vi "Digit to Color Converter.vi"(4 "Digit select":T1) -> (1 "Digit Color":u32(colorbox))   [LabVIEW 2018, in "Resistance Colors.lvlib"]
doc: "Converts the selected Digit Enum value into the corresponding color for the resistor band.\n\nThe VI receives the <b>Digit select</b> input and returns the corresponding resistor band color through <b>Digit Color</b>.\n\nThe color is determined by mapping the selected Enum item to the corresponding color constant."
uses:
  Resistance Colors.lvlib
  Resistor Controls/Digit--enum.ctl
  Band Colors/Band Colors.lvlib
  Resistor Controls/Resistance Controls.lvlib
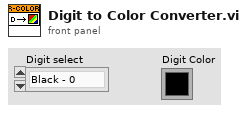
[diagram p1: front panel]
types:
  T1 = typedef "Resistance Controls.lvlib/Digit--enum.ctl" = enum16{"Black - 0", "Brown - 1", "Red - 2", "Orange - 3", "Yellow - 4", "Green - 5", "Blue - 6", "Violet - 7", "Grey - 8", "White - 9"}
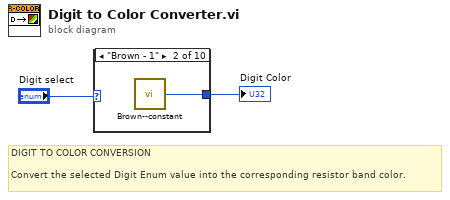
[diagram p0: block diagram]
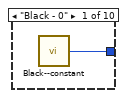
[diagram p2: hidden frame]
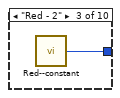
[diagram p3: hidden frame]
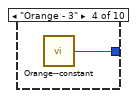
[diagram p4: hidden frame]
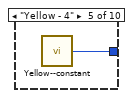
[diagram p5: hidden frame]
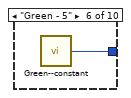
[diagram p6: hidden frame]
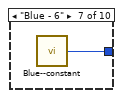
[diagram p7: hidden frame]
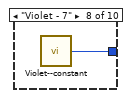
[diagram p8: hidden frame]
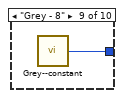
[diagram p9: hidden frame]
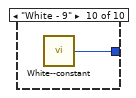
[diagram p10: hidden frame]
diagram:
  # "DIGIT TO COLOR CONVERSION\n\nConvert the selected Digit Enum value into the corresponding resistor band color."
  n1 = case shown="\"Brown - 1\"" "Digit select" {
    tunnel: [w3 w4 w5 w6 w7 w8 w9 w10 w11 w12] -> w1
    frame "Black - 0" {
      n2 = call "Black--constant.vi"() -> ("Black"=w3:u32)  [unwired: 5 in]
    }
    frame "Brown - 1" {
      n3 = call "Brown--constant.vi"() -> ("Brown"=w4:u32)  [unwired: 5 in]
    }
    frame "Red - 2" {
      n4 = call "Red--constant.vi"() -> ("Red"=w5:u32)  [unwired: 5 in]
    }
    frame "Orange - 3" {
      n5 = call "Orange--constant.vi"() -> ("Orange"=w6:u32)  [unwired: 5 in]
    }
    frame "Yellow - 4" {
      n6 = call "Yellow--constant.vi"() -> ("Yellow"=w7:u32)  [unwired: 5 in]
    }
    frame "Green - 5" {
      n7 = call "Green--constant.vi"() -> ("Green"=w8:u32)  [unwired: 5 in]
    }
    frame "Blue - 6" {
      n8 = call "Blue--constant.vi"() -> ("Blue"=w9:u32)  [unwired: 5 in]
    }
    frame "Violet - 7" {
      n9 = call "Violet--constant.vi"() -> ("Violet"=w10:u32)  [unwired: 5 in]
    }
    frame "Grey - 8" {
      n10 = call "Grey--constant.vi"() -> ("Gray"=w11:u32)  [unwired: 5 in]
    }
    frame "White - 9" {
      n11 = call "White--constant.vi"() -> ("White"=w12:u32)  [unwired: 5 in]
    }
  }
  "Digit Color" <- w1
